vi "Configure TS Panel.vi"(8 "error in (no error)":errorcluster, 11 "Generic Test Stand in":refnum<class "Generic Test Stand.lvclass">) -> (0 "error out":errorcluster, 3 "Generic Test Stand out":refnum<class "Generic Test Stand.lvclass">)   [LabVIEW 2019, in "Generic Test Stand.lvclass"]
uses:
  Generic Test Stand.lvclass
  Generic Test Stand.lvclass/Generic Test Stand.ctl
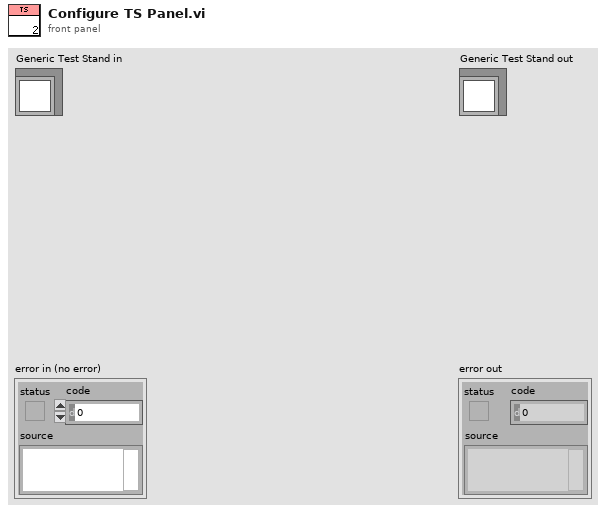
[diagram p1: front panel]
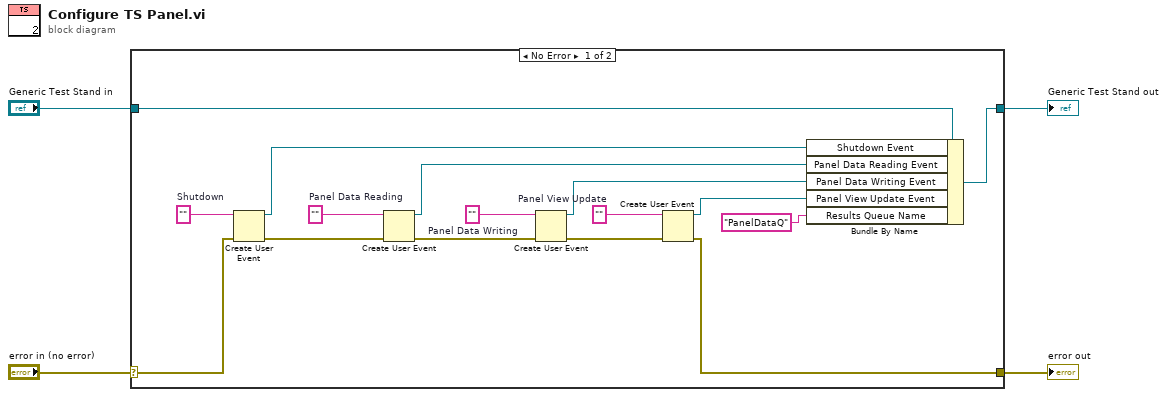
[diagram p0: block diagram]
diagram:
  n1 = case shown="No Error" "error in (no error)" {
    selector: "error in (no error)" -> [w13 w22]
    tunnel: [w5 w22] -> w3
    tunnel: [w10 w21] -> w1
    tunnel: "Generic Test Stand in" -> [w20 w21]
    frame No Error {
      w8 = ""  # Panel View Update
      w17 = ""  # Panel Data Writing
      w18 = ""  # Panel Data Reading
      w19 = ""  # Shutdown
      n2 = Create User Event(user event datatype=w19, error in=w13) -> (user event=w16:refnum<user-event>, error out=w12:errorcluster)
      n3 = Create User Event(user event datatype=w18, error in=w12) -> (user event=w15:refnum<user-event>, error out=w11:errorcluster)
      n4 = Create User Event(user event datatype=w17, error in=w11) -> (user event=w14:refnum<user-event>, error out=w6:errorcluster)
      n5 = Create User Event(user event datatype=w8, error in=w6) -> (user event=w7:refnum<user-event>, error out=w5:errorcluster)
      n6 = Bundle By Name(cluster=w20, "Shutdown Event"=w16, "Panel Data Reading Event"=w15, "Panel Data Writing Event"=w14, "Panel View Update Event"=w7, "Results Queue Name"="PanelDataQ" ("name (unnamed)")) -> (w10:refnum<class "Generic Test Stand.lvclass">)
    }
    frame Error {
    }
  }
  "error out" <- w3
  "Generic Test Stand out" <- w1
